vi "meas_osc_RS_2021.vi"() -> ()   [LabVIEW 2019]
uses:
  <instrlib>/Rohde&Schwarz RTx Oscilloscopes/Rohde&Schwarz RTx Oscilloscopes.lvlib
panel:
  out "Waveform Graph":dbl[](graph)
  in  "Time Base Range (0.5)":dbl=0.5 caption="Time Per Record (0.5)" format="%.3e"
  in  "Channel (1) 2":i32(ring)=1 caption="Channel (1)" items=["1"=1, "2"=2, "3"=3, "4"=4, "External"=5]
  in  "Vertical Coupling (DC 1 MOhm)":i32(ring) items=["AC", "DC 50 Ohm", "DC 1 MOhm", "AC 1 MOhm", "Ground"]
  in  "Vertical Range (0.04)":dbl=0.04 format="%.3e"
  out "Measurement Result":dbl format="%^.3e"
  in  "Measurement Function (Frequency)":i32(ring)=1 items=["Frequency"=1, "Period"=2, "Peak Peak"=3, "Peak Upper"=4, "Peak Lower"=5, "Positive Pulses Count"=6, "Negative Pulses Count"=7, "Rising Edges Count"=8, "Falling Edges Count"=9, "High"=10, "Low"=11, "Amplitude"=12, "Mean Value"=13, "RMS Value"=14, "Rise Time"=15, "Falling Time"=16, "Duty Cycle Positive"=17, "Duty Cycle Negative"=18, "Pulse Width Positive"=19, "Pulse Width Negative"=20, "Cycle Mean"=21, "Cycle RMS"=22, "Standard Deviation"=23, "Delay"=26, "Phase"=27, "Burst Width"=28, "Cycle Standard Deviation"=29, "Positive Overshoot"=30, "Negative Overshoot"=31]
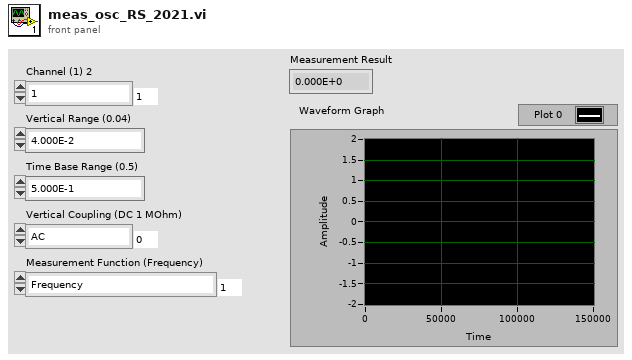
[diagram p1: front panel]
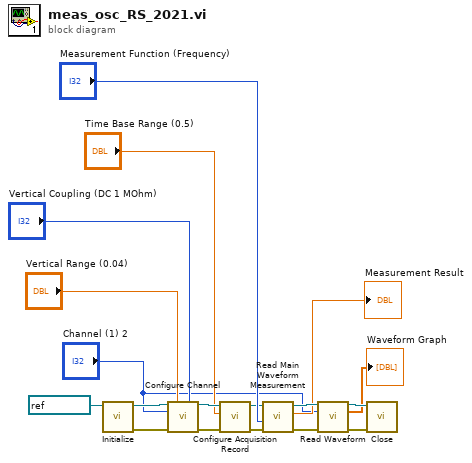
[diagram p0: block diagram]
diagram:
  n1 = call <instrlib>:"Initialize.vi"("VISA resource name"=refnum<visa-resource-name> "Rhode") -> ("error out"=w8:errorcluster, "VISA resource name out"=w9:refnum<visa-resource-name>)  [unwired: 9 in]
  n2 = call <instrlib>:"Configure Channel.vi"("VISA resource name"=w9, "Vertical Range (0.04)"="Vertical Range (0.04)", "Vertical Coupling (DC 1 MOhm)"="Vertical Coupling (DC 1 MOhm)", "Channel (1)"="Channel (1) 2", "error in (no error)"=w8) -> ("VISA resource name out"=w7:refnum<visa-resource-name>, "error out"=w6:errorcluster)  [unwired: 9 in]
  n3 = call <instrlib>:"Configure Acquisition Record.vi"("error in (no error)"=w6, "Time Per Record (0.5)"="Time Base Range (0.5)", "VISA resource name"=w7) -> ("error out"=w5:errorcluster, "VISA resource name out"=w4:refnum<visa-resource-name>)  [unwired: 7 in]
  n4 = call <instrlib>:"Read Main Waveform Measurement.vi"("error in (no error)"=w5, "Measurement Function (Frequency)"="Measurement Function (Frequency)", "VISA resource name"=w4) -> ("error out"=w16:errorcluster, "Measurement Result"=→"Measurement Result":dbl, "VISA resource name out"=w17:refnum<visa-resource-name>)  [unwired: 6 in]
  n5 = call <instrlib>:"Read Waveform.vi"("VISA resource name"=w17, "Channel (1)"="Channel (1) 2", "error in (no error)"=w16) -> ("VISA resource name out"=w13:refnum<visa-resource-name>, "Waveform Array"=→"Waveform Graph":dbl[], "error out"=w12:errorcluster)  [unwired: 7 in, 3 out]
  n6 = call <instrlib>:"Close.vi"("error in (no error)"=w12, "VISA resource name"=w13) -> ()  [unwired: 9 in, 1 out]
